vi "WriteDO.vi"(7 "GroveConnector":enum16{"D16", "D18", "D20"}(ring), 8 "error in (no error)":errorcluster, 9 "DO Value 2 (True)":bool, 10 "DO Value 1 (True)":bool, 11 "Session in":refnum<class "Session.lvclass">) -> (0 "error out":errorcluster, 3 "Session Out":refnum<class "Session.lvclass">)   [LabVIEW 2020]
doc: "Establishes communication with the instrument and optionally performs an instrument identification query and/or an instrument reset. It also places the instrument in a default state needed for other instrument driver operations. Therefore, call this VI before calling other instrument driver VIs for this instrument. Generally, you need to call the <b>Initialize</b> VI only once at the beginning of an application."
uses:
  CTI/Session/Session.lvclass
  CTI/GPIO Direction.ctl
  CTI/GPIO Number.ctl
  CTI/CTI.lvlib
panel:
  # "Input"
  # "Output"
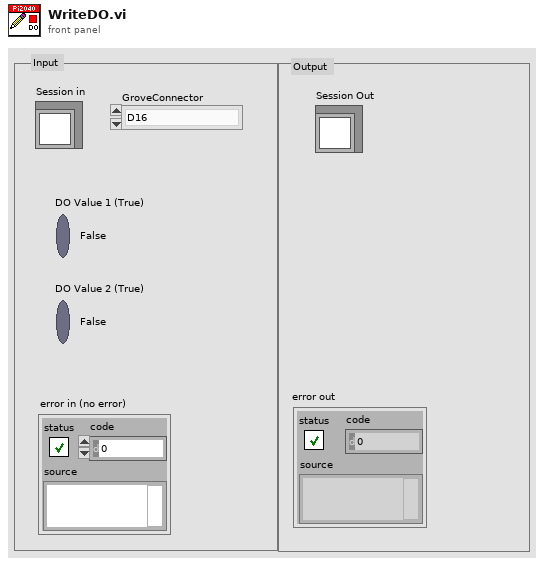
[diagram p1: front panel]
types:
  T1 = typedef "CTI.lvlib/GPIO Direction.ctl" = enum16{"In", "Out"}
  T2 = typedef "CTI.lvlib/GPIO Number.ctl" = i8
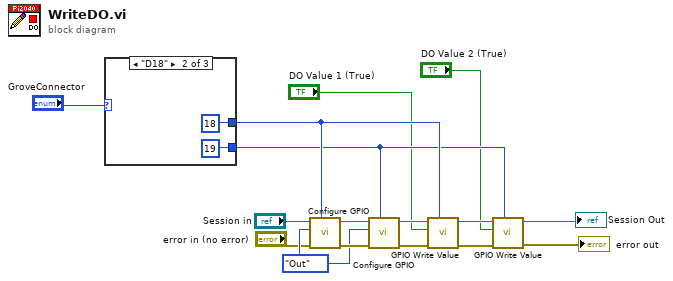
[diagram p0: block diagram]
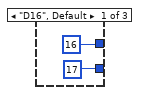
[diagram p2: hidden frame]
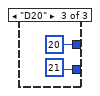
[diagram p3: hidden frame]
diagram:
  w14 = GPIO_Direction."Out" ("GPIO Direction")
  n1 = case shown="\"D18\"" "GroveConnector" {
    tunnel: [T2 16 ("GPIO #") T2 18 ("GPIO #") T2 20 ("GPIO #")] -> w11
    tunnel: [T2 17 ("GPIO #") T2 19 ("GPIO #") T2 21 ("GPIO #")] -> w8
    frame "D16", Default {
    }
    frame "D18" {
    }
    frame "D20" {
    }
  }
  n2 = call "Configure GPIO.vi"("GPIO #"=w11, "error in (no error)"="error in (no error)", "GPIO Direction"=w14, "Session in"="Session in") -> ("error out"=w15:errorcluster, "Session out"=w3:refnum<class "Session.lvclass">)  [unwired: 6 in]
  n3 = call "Configure GPIO.vi"("GPIO #"=w8, "error in (no error)"=w15, "GPIO Direction"=w14, "Session in"=w3) -> ("error out"=w12:errorcluster, "Session out"=w13:refnum<class "Session.lvclass">)  [unwired: 6 in]
  n4 = call "GPIO Write Value.vi"("GPIO #"=w11, "error in (no error)"=w12, "Value"="DO Value 1 (True)", "Session in"=w13) -> ("error out"=w9:errorcluster, "Session out"=w10:refnum<class "Session.lvclass">)  [unwired: 6 in]
  n5 = call "GPIO Write Value.vi"("GPIO #"=w8, "error in (no error)"=w9, "Value"="DO Value 2 (True)", "Session in"=w10) -> ("error out"=→"error out":errorcluster, "Session out"=→"Session Out":refnum<class "Session.lvclass">)  [unwired: 6 in]
